vi "Filter Controls and Indicators.vi"(0 "Controls[]":refnum<vi>[](array[refnum]), 11 "error in (no error)":errorcluster) -> (4 "Controls[]":refnum<vi>[](array[refnum]), 6 "Indicators[]":refnum<vi>[](array[refnum]), 15 "error out":errorcluster)   [LabVIEW 2021, in "Migrator.lvlib"]
uses:
  Migrator.lvlib
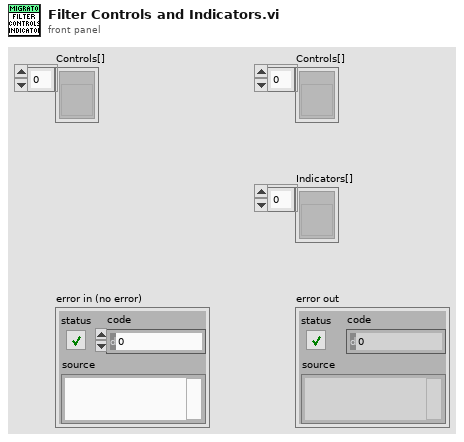
[diagram p1: front panel]
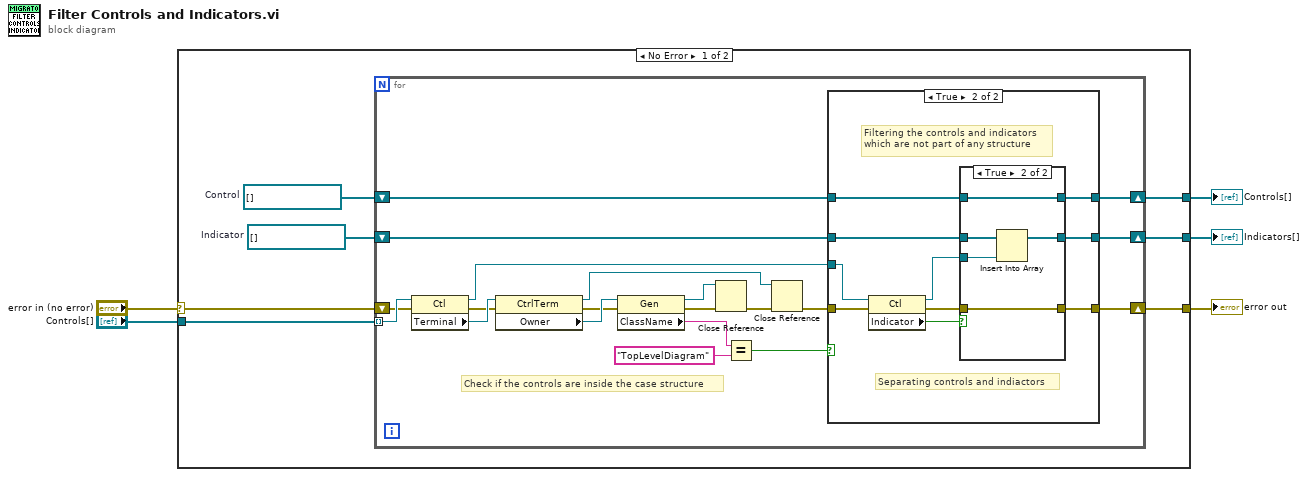
[diagram p0: block diagram]
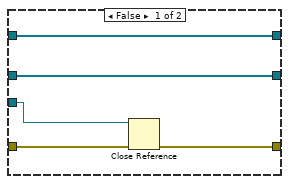
[diagram p2: hidden frame]
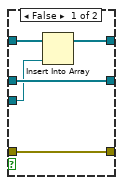
[diagram p3: hidden frame]
diagram:
  n1 = case shown="No Error" "error in (no error)" {
    selector: "error in (no error)" -> [w7 w58]
    tunnel: [w12 _] -> w5
    tunnel: [w11 _] -> w4
    tunnel: [w10 w58] -> w3
    tunnel: "Controls[]" -> [w6 _]
    frame No Error {
      w9 = refnum<vi>[] []  # Indicator
      w8 = refnum<vi>[] []  # Control
      n2 = for {
        tunnel: w6 -> [w32] mode=indexing
        shift-right: [w17] -> w10
        shift-left: w7 -> [w31]
        shift-right: [w19] -> w11
        shift-left: w8 -> [w21]
        shift-right: [w18] -> w12
        shift-left: w9 -> [w20]
        # "Check if the controls are inside the case structure"
        n3 = property class="Ctl"(reference=w32, error in=w31) -> (reference out=w22:refnum<vi>, error out=w28:errorcluster, "Terminal"=w30:refnum<vi>)
        n4 = property class="CtrlTerm"(reference=w30, error in=w28) -> (reference out=w13:refnum<vi>, error out=w27:errorcluster, "Owner"=w29:refnum<vi>)
        n5 = property class="Gen"(reference=w29, error in=w27) -> (reference out=w15:refnum<vi>, error out=w23:errorcluster, "ClassName"=w26:string)
        n6 = Close Reference(reference=w15, error in (no error)=w23) -> (error out=w16:errorcluster)
        n7 = Equal?(x=w26, y="TopLevelDiagram") -> (x = y?=w24:bool)
        n8 = Close Reference(reference=w13, error in (no error)=w16) -> (error out=w14:errorcluster)
        n9 = case shown="True" w24 {
          tunnel: w14 -> [w37 w46]
          tunnel: w22 -> [w33 w47]
          tunnel: w21 -> [w35 w43]
          tunnel: w20 -> [w36 w42]
          tunnel: [w35 w39] -> w19
          tunnel: [w36 w40] -> w18
          tunnel: [w34 w38] -> w17
          frame False {
            n10 = Close Reference(reference=w33, error in (no error)=w37) -> (error out=w34:errorcluster)
          }
          frame True {
            # "Separating controls and indiactors"
            # "Filtering the controls and indicators\nwhich are not part of any structure"
            n11 = property class="Ctl"(reference=w47, error in=w46) -> (reference out=w41:refnum<vi>, error out=w44:errorcluster, "Indicator"=w45:bool)
            n12 = case shown="True" w45 {
              tunnel: w44 -> [w48 w53]
              tunnel: w43 -> [w51 w54]
              tunnel: w42 -> [w52 w57]
              tunnel: w41 -> [w50 w56]
              tunnel: [w52 w55] -> w40
              tunnel: [w49 w54] -> w39
              tunnel: [w48 w53] -> w38
              frame False {
                n13 = Insert Into Array(array=w51, new element=w50) -> (w49:refnum<vi>[])  [unwired: 1 in]
              }
              frame True {
                n14 = Insert Into Array(array=w57, new element=w56) -> (w55:refnum<vi>[])  [unwired: 1 in]
              }
            }
          }
        }
      }
    }
    frame Error {
    }
  }
  "Indicators[]" <- w5
  "Controls[]" <- w4
  "error out" <- w3
